vi "SetFrequency.vi"(8 "error in (no error)":errorcluster, 10 "Freq":sgl[](array[numeric]), 11 "I2C PWM in":refnum<class "I2C PWM.lvclass">) -> (0 "error out":errorcluster, 3 "I2C PWM out":refnum<class "I2C PWM.lvclass">)   [LabVIEW 2020, in "CTI-Peripheral.lvlib" / "I2C PWM.lvclass"]
uses:
  I2C PWM.lvclass
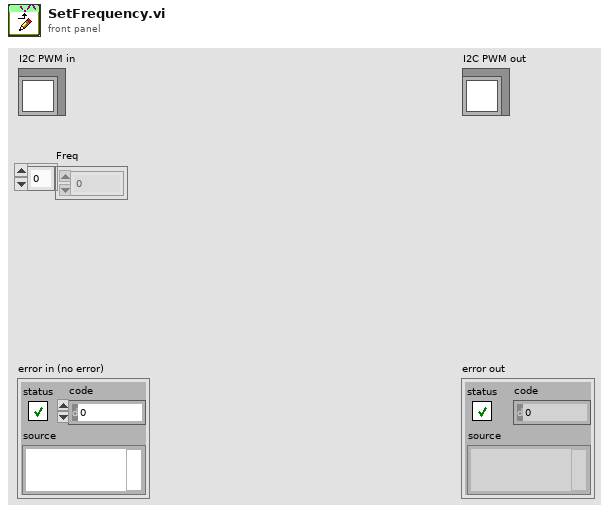
[diagram p1: front panel]
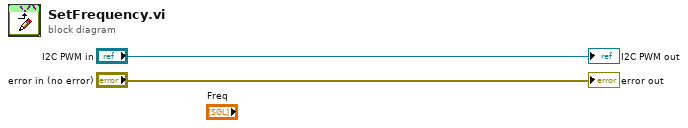
[diagram p0: block diagram]
diagram:
  "error out" <- "error in (no error)"
  "I2C PWM out" <- "I2C PWM in"
